vi "MTD_MathScript.vi"(0 "MTD Input":cdb[](array[numeric]), 1 "NFFT":i32, 2 "NPRI":i32, 3 "PRF":i32) -> (7 "MTD Output":cdb[](array[numeric]), 9 "MTD_Max":cdb[](array[numeric]), 10 "Max_Index":dbl[](array[numeric]))   [LabVIEW 2012]
uses:
  <vilib>/imath/engines/lvmath/Plug In/_Char/NIMS_CH_character datatype.ctl
  <vilib>/imath/engines/lvmath2/RunTimeEngine/ErrorHandling/NIMS_Finalize Error.vi
  <vilib>/imath/engines/lvmath/Plug In/_Char/NIMS_CH_Character RV to String.vi
  <vilib>/imath/engines/lvmath2/RunTimeEngine/BuiltInFunctions/error/NIMS_error.vi
  <vilib>/imath/engines/lvmath2/RunTimeEngine/NodeEndStatement/NIMS_NodeEndStatement_Output.vi
  <instcachedir>/0/NIMS_NodeEndStatement_Output_53EC0D466D134D7ABD903AC30B43404B.lvgen/NIMS_NodeEndStatement_Output_53EC0D466D134D7ABD903AC30B43404B_005.vi
  <instcachedir>/0/NIMS_NodeEndStatement_Output_53EC0D466D134D7ABD903AC30B43404B.lvgen/NIMS_NodeEndStatement_Output_53EC0D466D134D7ABD903AC30B43404B_000.vi
  <instcachedir>/0/NIMS_NodeEndStatement_Output_53EC0D466D134D7ABD903AC30B43404B.lvgen/NIMS_NodeEndStatement_Output_53EC0D466D134D7ABD903AC30B43404B_012.vi
  <vilib>/imath/engines/lvmath2/RunTimeEngine/BuiltInFunctions/zeros/NIMS_V=zeros(I32,I32).vi
  <vilib>/imathl/engines/lvmath/Functions/Error Handling/Create Error.vi
  <vilib>/imath/engines/lvmath2/RunTimeEngine/BuiltInFunctions/zeros/NIMS_M=zeros(I32,I32).vi
  <vilib>/imath/engines/lvmath2/RunTimeEngine/RangeToken/NIMS_Range_R2 - Integer.vi
  <instcachedir>/0/NIMS_Range_R2 - Integer_CD92A44154CA48D58B2F3E711AB114DB.lvgen/NIMS_Range_R2 - Integer_CD92A44154CA48D58B2F3E711AB114DB_000.vi
  <vilib>/imath/engines/lvmath2/RunTimeEngine/CommandStatement/MC_CommandStatement_break.vi
  <vilib>/imath/engines/lvmath2/RunTimeEngine/ReplaceToken/NIMS_Replace - Check Row.vi
  <instcachedir>/0/NIMS_Replace - Check Row_8C35B66FE73A429EAC382AAA935851F0.lvgen/NIMS_Replace - Check Row_8C35B66FE73A429EAC382AAA935851F0_006.vi
  <vilib>/imath/engines/lvmath2/RunTimeEngine/ReplaceToken/NIMS_Replace - Check Column.vi
  <instcachedir>/0/NIMS_Replace - Check Column_F9ADE87E459D46779ACFAE3AFB317B9B.lvgen/NIMS_Replace - Check Column_F9ADE87E459D46779ACFAE3AFB317B9B_003.vi
  <vilib>/imath/engines/lvmath2/RunTimeEngine/VariableToken/Read/NIMS_Get Elements - RV(_) - Check.vi
  <instcachedir>/0/NIMS_Get Elements - RV(_) - Check_09E565EE58C54071A799578B82C9999A.lvgen/NIMS_Get Elements - RV(_) - Check_09E565EE58C54071A799578B82C9999A_005.vi
  <vilib>/imath/engines/lvmath2/RunTimeEngine/ReplaceToken/NIMS_Replace - Size Check M(_,_)=S.vi
  <instcachedir>/0/NIMS_Replace - Size Check M(_,_)=S_0CFA00F12BB840EDA61E43D782562782.lvgen/NIMS_Replace - Size Check M(_,_)=S_0CFA00F12BB840EDA61E43D782562782_001.vi
  <vilib>/imath/engines/lvmath2/RunTimeEngine/ReplaceToken/NIMS_Replace - M(S,S)=S.vi
  <instcachedir>/0/NIMS_Replace - M(S,S)=S_59120E3D3E804D63A1B2B7FDD4B95F55.lvgen/NIMS_Replace - M(S,S)=S_59120E3D3E804D63A1B2B7FDD4B95F55_001.vi
  <vilib>/imath/engines/lvmath2/RunTimeEngine/ErrorHandling/NIMS_Create Error From Enums.vi
  <vilib>/imath/engines/lvmath2/RunTimeEngine/VariableToken/Read/NIMS_Get Elements - SorM(_,$) - Check.vi
  <instcachedir>/0/NIMS_Get Elements - SorM(_,$) - Check_FE352FA85B844FB785E5C28FDABD92A5.lvgen/NIMS_Get Elements - SorM(_,$) - Check_FE352FA85B844FB785E5C28FDABD92A5_002.vi
  <vilib>/imath/engines/lvmath2/RunTimeEngine/BuiltInFunctions/fft/NIMS_fft(GV).vi
  <instcachedir>/0/NIMS_fft(GV)_4C6467FC22F84E4BA42517A07EF978B0.lvgen/NIMS_fft(GV)_4C6467FC22F84E4BA42517A07EF978B0_001.vi
  <vilib>/imath/engines/lvmath2/RunTimeEngine/ReplaceToken/NIMS_Replace - Size Check M(_,$)=VorM.vi
  <instcachedir>/0/NIMS_Replace - Size Check M(_,$)=VorM_05C8DDF28A13406EBCBD8C1ACDF4F548.lvgen/NIMS_Replace - Size Check M(_,$)=VorM_05C8DDF28A13406EBCBD8C1ACDF4F548_011.vi
  <vilib>/imath/engines/lvmath2/RunTimeEngine/ReplaceToken/NIMS_Replace - Assignment Check M(_,$)=VorM.vi
  <instcachedir>/0/NIMS_Replace - Assignment Check M(_,$)=VorM_DBF82BC42B054E2BA4F8E4D1989751AD.lvgen/NIMS_Replace - Assignment Check M(_,$)=VorM_DBF82BC42B054E2BA4F8E4D1989751AD_011.vi
  <vilib>/imath/engines/lvmath2/RunTimeEngine/BuiltInFunctions/max/1 input/NIMS_max(CV).vi
  <instcachedir>/0/NIMS_max(CV)_AC556B0302EC458D9C500E1D551C3BD8.lvgen/NIMS_max(CV)_AC556B0302EC458D9C500E1D551C3BD8_000.vi
  <vilib>/imath/engines/lvmath2/RunTimeEngine/ReplaceToken/NIMS_Replace - Check Linear.vi
  <instcachedir>/0/NIMS_Replace - Check Linear_44ABB4D6A819426DBDF25CCE6827BF1D.lvgen/NIMS_Replace - Check Linear_44ABB4D6A819426DBDF25CCE6827BF1D_002.vi
  <vilib>/imath/engines/lvmath2/RunTimeEngine/ReplaceToken/NIMS_Replace - Size Check _(_)=S.vi
  <instcachedir>/0/NIMS_Replace - Size Check _(_)=S_5AC8AA27B9694BB9828B57BCF666F597.lvgen/NIMS_Replace - Size Check _(_)=S_5AC8AA27B9694BB9828B57BCF666F597_001.vi
  <vilib>/imath/engines/lvmath2/RunTimeEngine/ReplaceToken/NIMS_Replace - V(S)=S.vi
  <instcachedir>/0/NIMS_Replace - V(S)=S_927EF1B21AA84780A9A306EC96B904EC.lvgen/NIMS_Replace - V(S)=S_927EF1B21AA84780A9A306EC96B904EC_001.vi
  <instcachedir>/0/NIMS_Replace - Check Linear_44ABB4D6A819426DBDF25CCE6827BF1D.lvgen/NIMS_Replace - Check Linear_44ABB4D6A819426DBDF25CCE6827BF1D_001.vi
  <instcachedir>/0/NIMS_Replace - Size Check _(_)=S_5AC8AA27B9694BB9828B57BCF666F597.lvgen/NIMS_Replace - Size Check _(_)=S_5AC8AA27B9694BB9828B57BCF666F597_000.vi
  <instcachedir>/0/NIMS_Replace - V(S)=S_927EF1B21AA84780A9A306EC96B904EC.lvgen/NIMS_Replace - V(S)=S_927EF1B21AA84780A9A306EC96B904EC_000.vi
  <vilib>/imath/engines/lvmath2/RunTimeEngine/RangeToken/NIMS_Range_R2.vi
  <instcachedir>/0/NIMS_Replace - Check Linear_44ABB4D6A819426DBDF25CCE6827BF1D.lvgen/NIMS_Replace - Check Linear_44ABB4D6A819426DBDF25CCE6827BF1D_000.vi
  <vilib>/imath/engines/lvmath2/RunTimeEngine/VariableToken/Read/NIMS_Get Elements - SorM(_,_) - Check - Check.vi
  <instcachedir>/0/NIMS_Get Elements - SorM(_,_) - Check - Check_3492346BAECA4EC09E2016EA7EC0034B.lvgen/NIMS_Get Elements - SorM(_,_) - Check - Check_3492346BAECA4EC09E2016EA7EC0034B_006.vi
  <vilib>/imath/engines/lvmath2/RunTimeEngine/ReplaceToken/NIMS_Replace - Size Check _(_)=VorM.vi
  <instcachedir>/0/NIMS_Replace - Size Check _(_)=VorM_9634A4AA7447414F8F7800030F26CE99.lvgen/NIMS_Replace - Size Check _(_)=VorM_9634A4AA7447414F8F7800030F26CE99_012.vi
  <vilib>/imath/engines/lvmath2/RunTimeEngine/ReplaceToken/NIMS_Replace - Assignment Check _(_)=VorM.vi
  <instcachedir>/0/NIMS_Replace - Assignment Check _(_)=VorM_B6C77D2C692B4FA588678A90042D4473.lvgen/NIMS_Replace - Assignment Check _(_)=VorM_B6C77D2C692B4FA588678A90042D4473_012.vi
panel:
  out "Input Size":i32
  out "PRF":i32
  out "NPRI":i32
  out "NFFT":i32
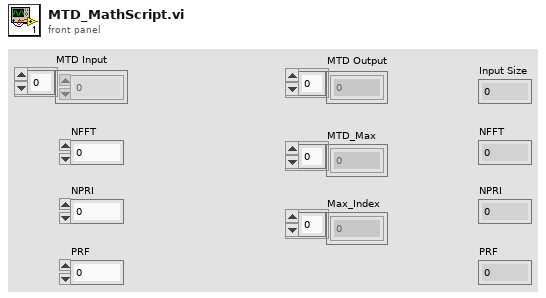
[diagram p1: front panel]
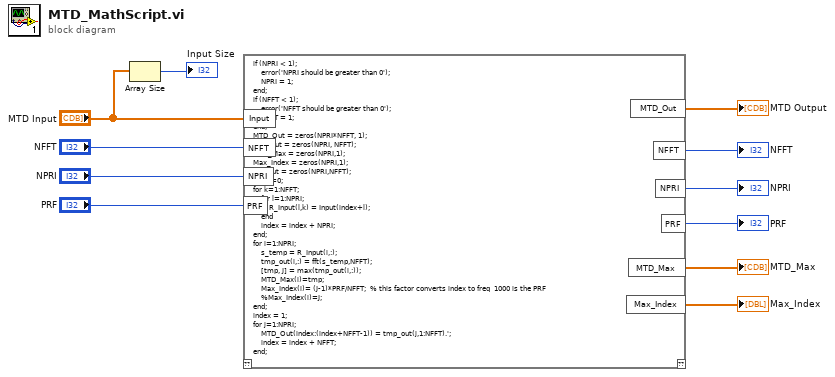
[diagram p0: block diagram]
diagram:
  n1 = Array Size(array="MTD Input") -> (size(s)=→"Input Size":i32)
  n2 = mathscript code="if (NPRI < 1);\n    error('NPRI should be greater than 0');\n    NPRI = 1;\nend;\nif (NFFT < 1);\n    error('NFFT should be greater than 0');\n    NFFT = 1;\nend;\nMTD_Out = zeros(NPRI*NFFT, 1);\ntmp_out = zeros(NPRI, NFFT);\nMTD_Max = zeros(NPRI,1);\nMax_Index = zeros(NPRI,1);\nR_Input = zeros(NPRI,NFFT);\nindex=0;\nfor k=1:NFFT;\n    for l=1:NPRI;\n        R_Input(l,k) = Input(index+l);\n    end\n    index = index + NPRI;\nend;\nfor i=1:NPRI;\n    s_temp = R_Input(i,:);\n    tmp_out(i,:) = fft(s_temp,NFFT);\n    [tmp, J] = max(tmp_out(i,:));\n    MTD_Max(i)=tmp;\n    Max_Index(i)= (J-1)*PRF/NFFT;  % this factor converts index to freq  1000 is the PRF\n    %Max_Index(i)=J;\nend;\nindex = 1;\nfor j=1:NPRI;\n    MTD_Out(index:(index+NFFT-1)) = tmp_out(j,1:NFFT).';\n    index = index + NFFT;\nend;"("Input"="MTD Input", "NFFT"="NFFT", "NPRI"="NPRI", "PRF"="PRF") -> ("MTD_Out"=→"MTD Output":dbl[], "NFFT"=→"NFFT":i32, "NPRI"=→"NPRI":i32, "PRF"=→"PRF":i32, "MTD_Max"=→"MTD_Max":cdb[], "Max_Index"=→"Max_Index":dbl[])  [unwired: 1 in, 1 out]
